vi "Creation_chemin.vi"(2 "Répertoire de travail":path) -> (0 "Chemin du fichier":path)   [LabVIEW 2022 SP3]
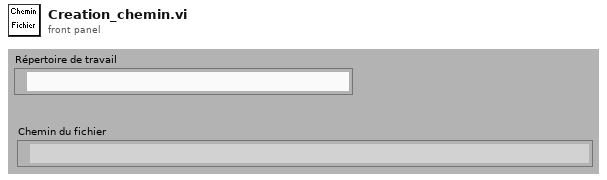
[diagram p1: front panel]
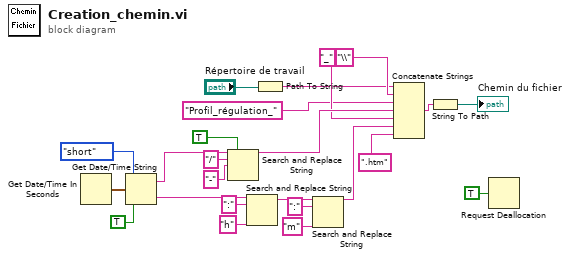
[diagram p0: block diagram]
diagram:
  n1 = Get Date/Time In Seconds() -> (seconds since 1Jan1904=w12:timestamp)
  n2 = Get Date/Time String(date format (0)=enum16{"short", "long", "abbreviated"}."short" ("format de date (0)"), seconds (now)=w12, want seconds? (F)=TRUE ("secondes ? (F)")) -> (date string=w17:string, time string=w22:string)
  n3 = Search and Replace String(replace all?=TRUE ("tout remplacer ? (F)"), input string=w17, search string="/" ("chaîne recherchée"), replace string="-" ("chaîne de remplacement (\"\")")) -> (result string=w19:string)  [unwired: 4 in, 3 out]
  n4 = Search and Replace String(input string=w22, search string=":" ("chaîne recherchée"), replace string="h" ("chaîne de remplacement (\"\")")) -> (result string=w2:string)  [unwired: 5 in, 3 out]
  n5 = Path To String(path="Répertoire de travail") -> (string=w10:string)
  n6 = Search and Replace String(input string=w2, search string=":" ("chaîne recherchée"), replace string="m" ("chaîne de remplacement (\"\")")) -> (result string=w3:string)  [unwired: 5 in, 3 out]
  n7 = Concatenate Strings(w10, "\\", "Profil_régulation_" ("chaîne"), w19, "_", w3, ".htm") -> (w8:string)
  n8 = String To Path(string=w8) -> (path=→"Chemin du fichier":path)
  n9 = Request Deallocation(TRUE ("flag")) -> ()
